vi "MQTT Client - Configure Will.vi"(0 "MQTT Session":T1, 1 "Will Retain (False)":bool, 5 "Will Topic":string, 7 "Will Payload":string, 9 "Will QoS (0)":u8, 11 "error in":errorcluster, 12 "WILL Properties (v5)":T2[](array[typedef]) {"Property" items=[" Payload Format Indicator          "=1, " Message Expiry Interval           "=2, " Content Type                      "=3, " Response Topic                    "=8, " Correlation Data                  "=9, " Will Delay Interval               "=24, " User Property                     "=38]}) -> (4 "MQTT Session out":T1, 15 "error out":errorcluster)   [LabVIEW 2019, in "KoRE-MQTT.lvlib"]
doc: "<b>Description:</b> This VI configures the \"Will\" message settings for an MQTT client session. It specifies parameters such as retention, topic, payload, and quality of service for messages sent when the client disconnects unexpectedly.\n\n<b>Input Terminals:</b>\n- <b>Will Retain (False) [1]</b>: Boolean value indicating whether the \"Will\" message should be retained by the broker after being delivered.\n- <b>MQTT Session [0]</b>: Reference to the MQTT session that will utilize the configured Will settings.\n- <b>MQTT Session [4]</b>: Reference to the MQTT session that will utilize the configured \"Will\" settings.\n- <b>Will Topic [5]</b>: The topic for the \"Will\" message that will be published upon an unexpected disconnection.\n- <b>Will Payload [7]</b>: The payload of the \"Will\" message, which will be sent to the specified topic when the client disconnects unexpectedly.\n- <b>Will QoS (0) [9]</b>: Quality of Service level for the \"Will\" message, dictating the delivery guarantee (0 for at most once, 1 for at least once, and 2 for exactly once).\n- <b>WILL Properties [12]</b>: Optional array of Property and Value pairs specifically applicable for MQTT v5 connections, allowing additional \"Will\" properties.\n\n<b>Output Terminals:</b>\n- <b>MQTT Session out [4] (v5) </b>: Reference to the configured MQTT session with the applied Will settings.\n\nCopyright (c) 2025 KoRElibs.com\nSPDX-License-Identifier: EUPL-1.2\n\nThis VI is licensed under the European Union Public License (EUPL) Version 1.2. You may use this VI unmodified in proprietary works. If you distribute a modified version of this file, the modified file must be released under the EUPL-1.2. Full license: https://joinup.ec.europa.eu/asset/eupl/eupl/1.2/"
uses:
  KoRE-MQTT.lvlib
  TypeDefs/MQTT Property - Will.ctl
  TypeDefs/MQTT Client Session.ctl
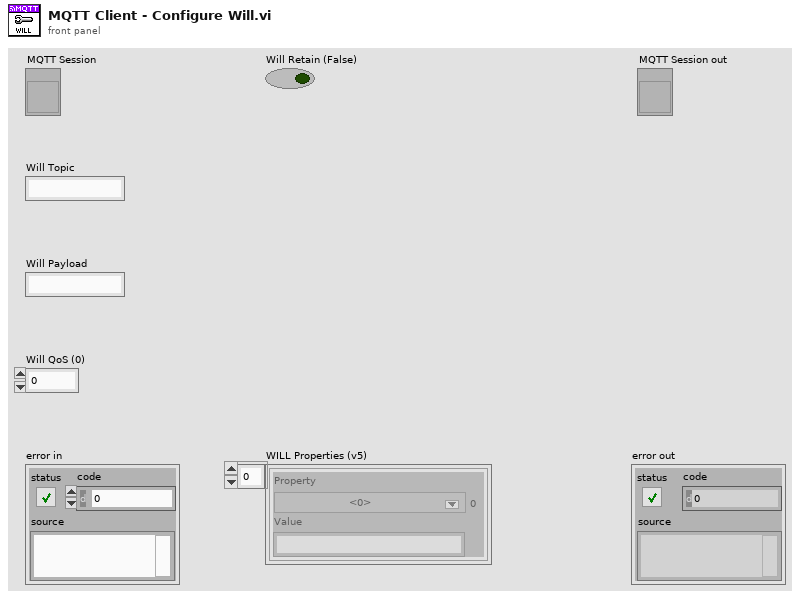
[diagram p1: front panel]
types:
  T1 = typedef "KoRE-MQTT.lvlib/MQTT Client Session.ctl" = refnum<vi>
  T2 = typedef "KoRE-MQTT.lvlib/MQTT Property - Will.ctl" = cluster{"Property":u8, "Value":string}
  T3 = typedef "KoRE-MQTT.lvlib/MQTT Client Session - Data.ctl" = cluster{"TCP ref":refnum<k5>, "Next Packet Id":u16, "Version":u8, "Host":string, "Port":u16, "Ping Delta":u32, "Username":string, "Password":string, "Will QoS":u8, "Will Retain":bool, "Will Topic":string, "Will Payload":string, "TCP Timeout":i32, "Semaphore":T4, "In-Flight Messages":variant, "Close":bool, "Last Send":u32, "Keep Alive":u16, "Last Ping RTT":u32, "Last Ping":u32, "Will Properties":T2[], "Session Expiry Interval":u32, "Maximum QoS":u8, "Retain Available":bool, "Server Maximum Packet Size":u32, "Client Identifier":string, "Server Topic Alias Maximum":u16, "Wildcard Subscription Available":bool, "Subscription Identifier Available":bool, "Shared Subscription Available":bool, "Connect Properties":T5[], "Client Maximum Packet Size":u32, "Client Topic Alias Maximum":u16, "Server Receive Maximum":u16, "Client Receive Maximum":u16, "TLS cfg":refnum<k36>, "Subscriptions":T6[]}
  T4 = typedef "Semaphore RefNum" = refnum<k1>
  T5 = typedef "KoRE-MQTT.lvlib/MQTT Property - CONNECT.ctl" = cluster{"Property":u8, "Value":string}
  T6 = typedef "KoRE-MQTT.lvlib/MQTT Subscription - Info.ctl" = cluster{"Packet Id":u16, "Index":u16, "Identifier":u32, "QoS":u8, "Topic Filter":string, "Reason Code":u8, "Reason String":string, "Granted":bool}
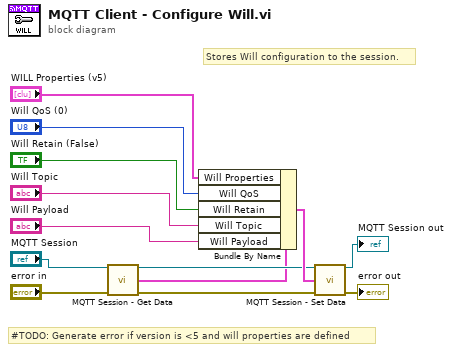
[diagram p0: block diagram]
diagram:
  # "Stores Will configuration to the session."
  # "#TODO: Generate error if version is <5 and will properties are defined"
  n1 = call "MQTT Session - Get Data.vi"("mqtt ref in"="MQTT Session", "error in"="error in") -> ("mqtt ref out"=w2:T1, "mqtt ref data"=w1:T3, "error out"=w5:errorcluster)  [unwired: 11 in]
  n2 = Bundle By Name(cluster=w1, "Will Properties"="WILL Properties (v5)", "Will QoS"="Will QoS (0)", "Will Retain"="Will Retain (False)", "Will Topic"="Will Topic", "Will Payload"="Will Payload") -> (w6:T3)
  n3 = call "MQTT Session - Set Data.vi"("mqtt ref in"=w2, "mqtt ref data"=w6, "error in"=w5) -> ("mqtt ref out"=→"MQTT Session out":T1, "error out"=→"error out":errorcluster)  [unwired: 11 in]
